vi "from string array.vi"(8 "error in (no error)":errorcluster, 9 "String Array":string[][](array[string]), 10 "version":string, 11 "module configuration in":refnum<class "Daqmx Module configuration.lvclass">) -> (0 "error out":errorcluster, 3 "module configuration out":refnum<class "Daqmx Module configuration.lvclass">)   [LabVIEW 2015, in "DAQmx Module Configuration.lvclass"]
uses:
  Daqmx Module configuration.lvclass
  Line.ctl
  <vilib>/NI/Tag Bus Module Framework/channel/TBM channel.lvclass
  Measurement Type.ctl
  Parameters.ctl
  <vilib>/NI/Tag Bus/tag/Data Type.ctl
  <vilib>/NI/Tag Bus Module Framework/channel/channel classification.ctl
  Daqmx Module configuration.lvclass/Daqmx Module configuration.ctl
  <vilib>/NI/Tag Bus/tag/tag descriptor.lvclass
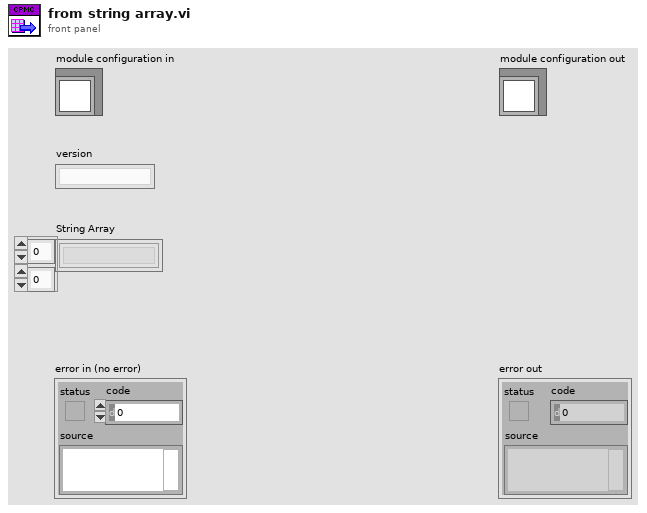
[diagram p1: front panel]
types:
  T1 = typedef "DAQmx Module Configuration.lvclass/Line.ctl" = cluster{"Channel Array":refnum<class "TBM channel.lvclass">[], "Physical Channel":string, "Measurement Type":T2, "Parameters":T3}
  T2 = typedef "DAQmx Module Configuration.lvclass/Measurement Type.ctl" = enum16{"Digital Input", "Digital Output", "Voltage Input", "Voltage Output", "Current Input", "Current Output", "RTD", "Thermocouple", "Strain", "PWM"}
  T3 = typedef "DAQmx Module Configuration.lvclass/Parameters.ctl" = cluster{"Digital Config":cluster{"Invert Lines?":bool}, "Voltage Config":cluster{"Maximum Value (V)":dbl, "Minimum Value (V)":dbl, "in terminal configuration (V)":i32, "out terminal configuration (V)":i32}, "Current Config":cluster{"Maximum Value (A)":dbl, "Minimum Value (A)":dbl, "shunt resistor location":i32, "input terminal configuration (C)":i32, "external shunt resistor value":dbl}, "RTD Config":cluster{"Maximum Value (°C)":dbl, "Minimum Value (°C)":dbl, "resistance configuration":i32, "r0":dbl, "current excitation value":dbl, "rtd type":i32, "current excitation source":i32}, "Thermocouple Config":cluster{"Minimum Value (C)":dbl, "Maximum Value (C)":dbl, "thermocouple type":i32, "cjc source":i32, "cjc value":dbl}, "Strain Config":cluster{"Maximum Value":dbl, "Minimum Value":dbl, "bridge information":cluster{"strain configuration":i32, "lead wire resistance":dbl, "initial bridge voltage":dbl, "voltage excitation source":i32, "voltage excitation value":dbl}, "strain gage information":cluster{"gage factor":dbl, "nominal gage resistance":dbl, "poisson ratio":dbl}}, "PWM Config":cluster{"Idle State":bool}}
  T4 = typedef "TBM channel.lvclass/channel classification.ctl" = enum16{"input data", "output data", "processing parameter", "processing result"}
  T5 = typedef "tag bus.lvlib/tag descriptor.lvclass/Data Type.ctl" = enum16{"Double", "Single", "I64", "I32", "I16", "I8", "U64", "U32", "U16", "U8", "Boolean", "String", "Array of Double", "Array of Single", "Array of I64", "Array of I32", "Array of I16", "Array of I8", "Array of U64", "Array of U32", "Array of U16", "Array of U8", "Array of Boolean", "Array of String"}
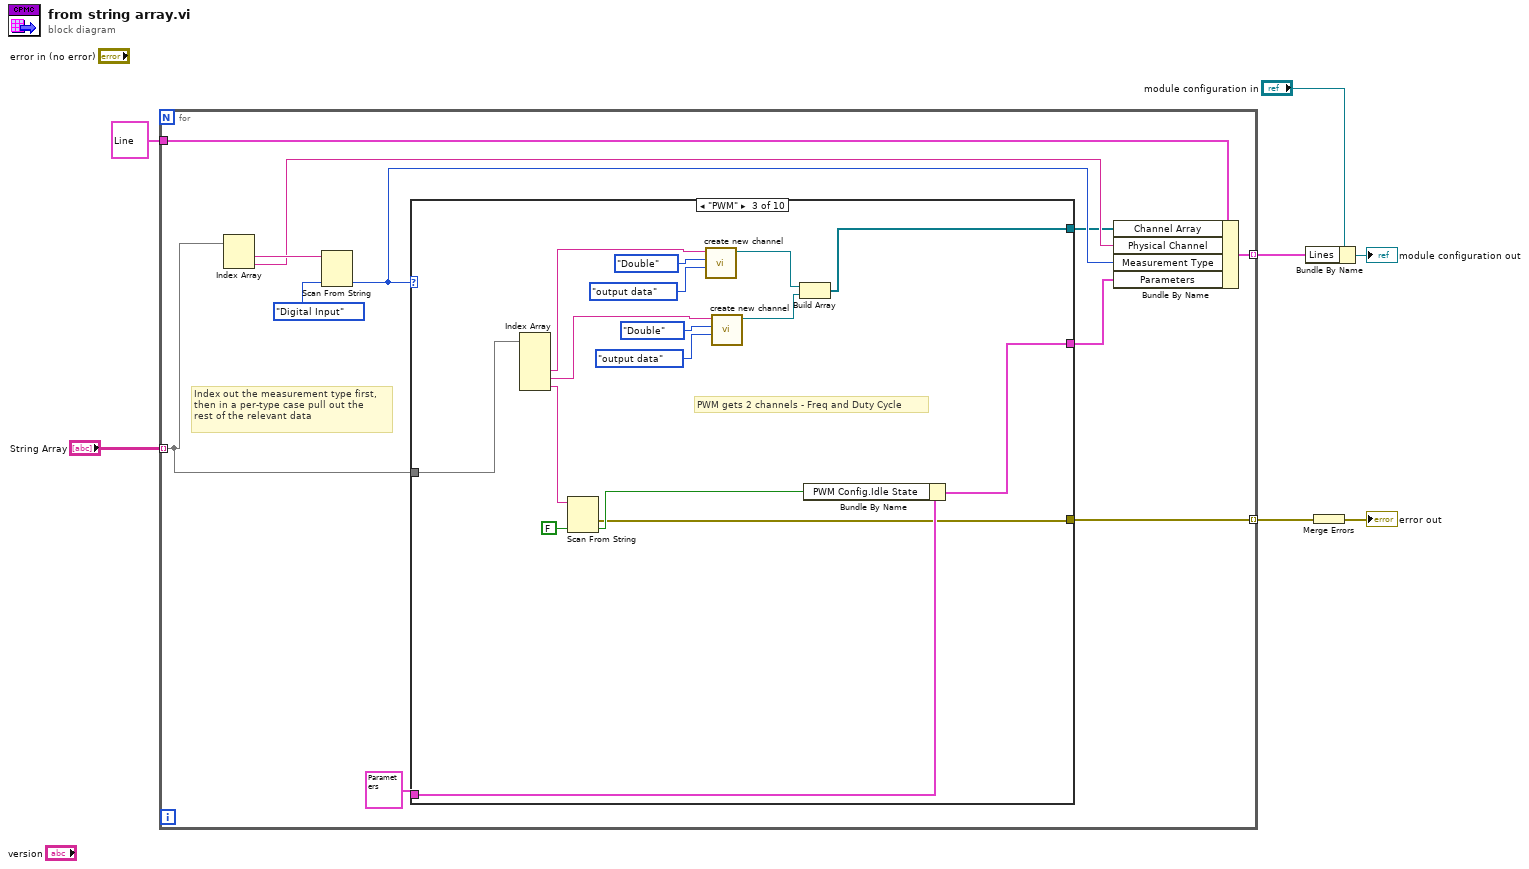
[diagram p0: block diagram]
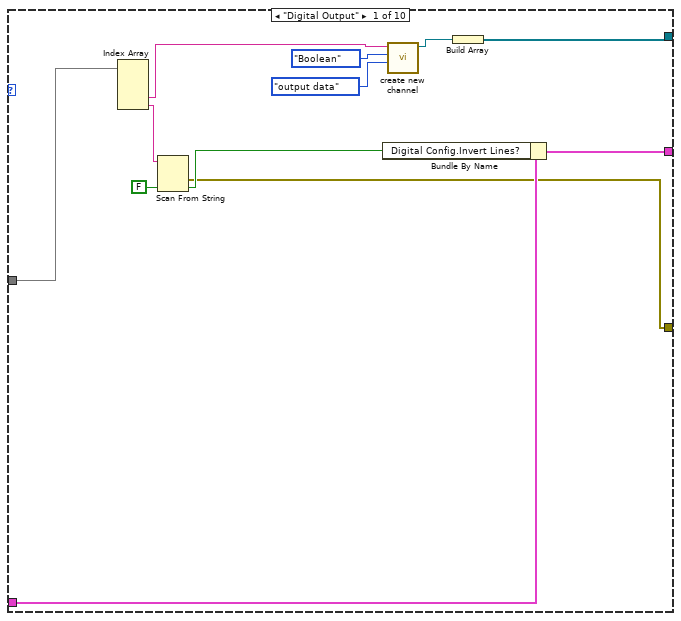
[diagram p2: hidden frame]
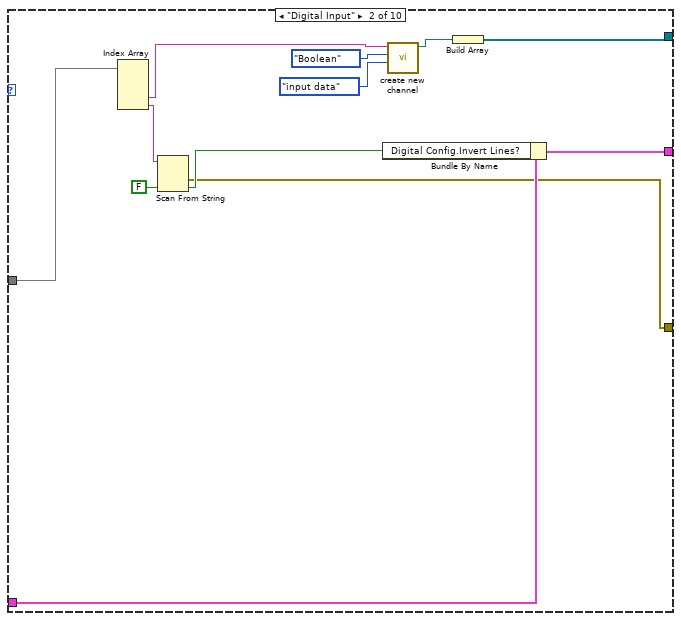
[diagram p3: hidden frame]
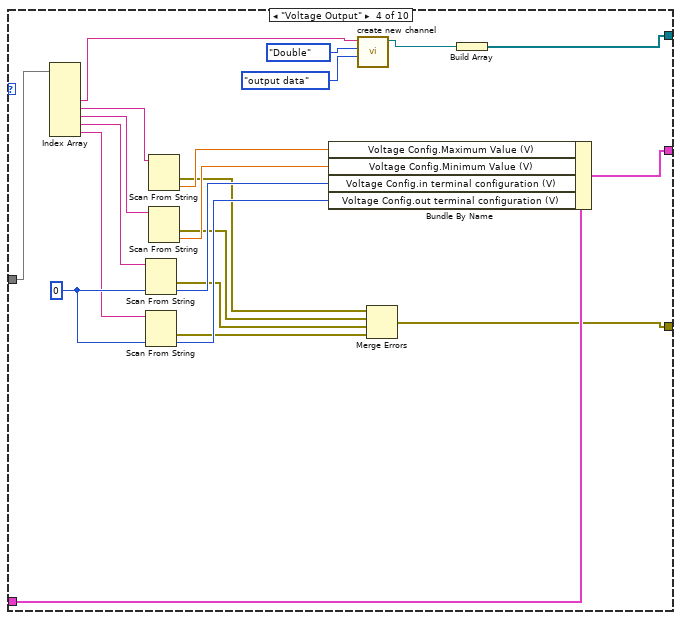
[diagram p4: hidden frame]
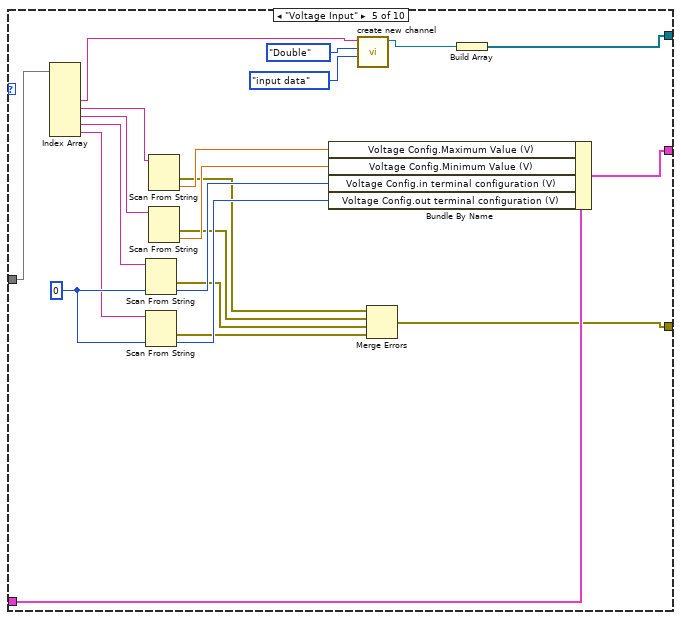
[diagram p5: hidden frame]
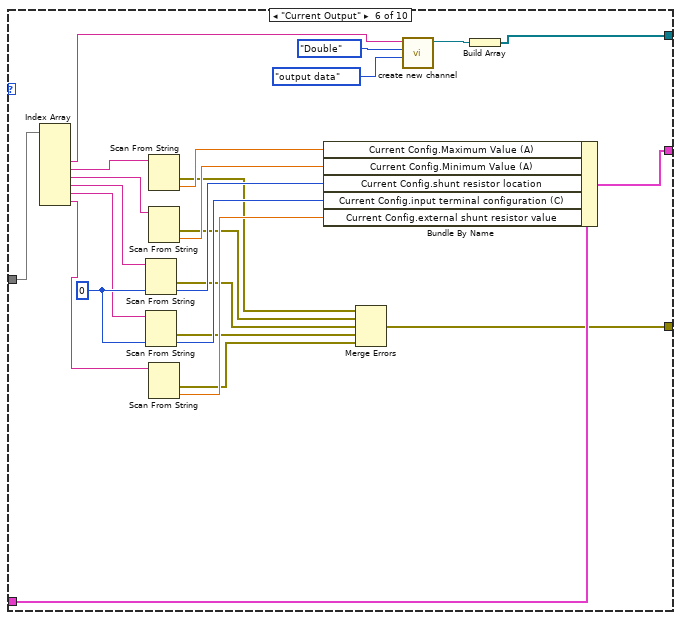
[diagram p6: hidden frame]
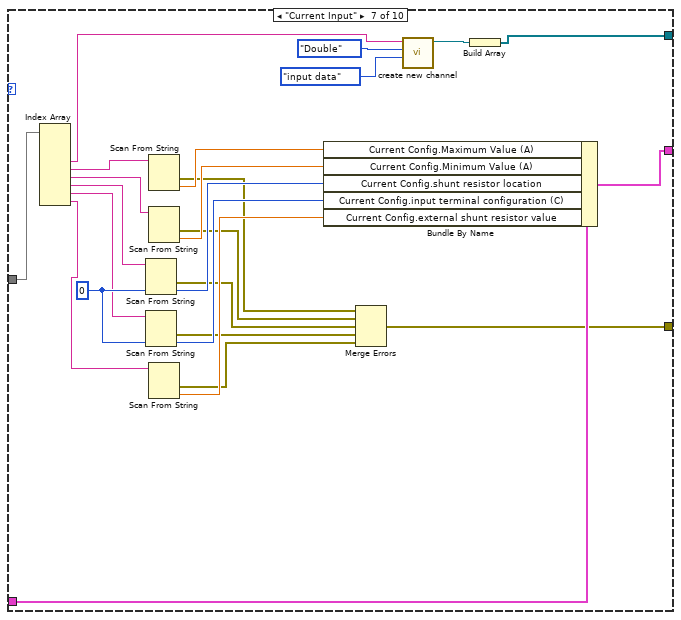
[diagram p7: hidden frame]
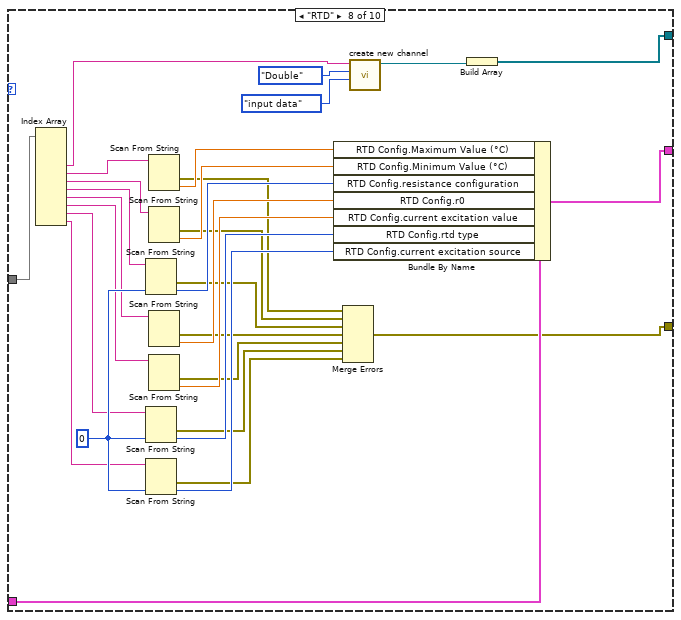
[diagram p8: hidden frame]
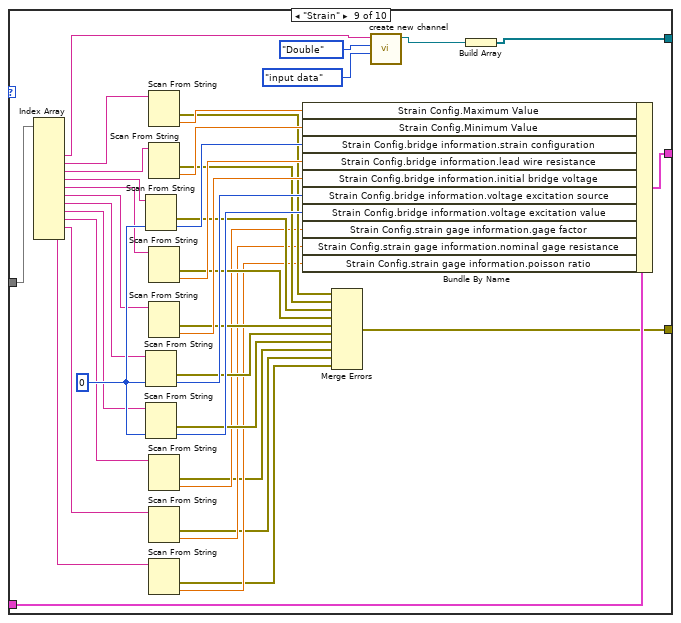
[diagram p9: hidden frame]
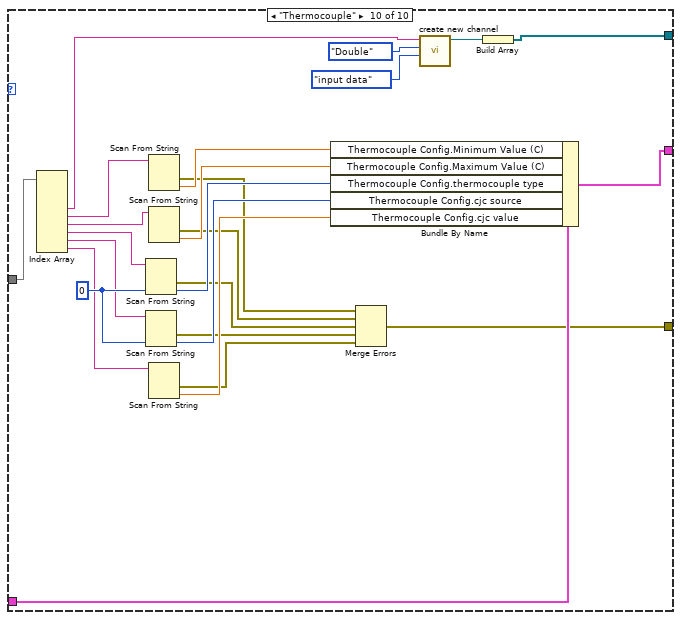
[diagram p10: hidden frame]
diagram:
  n1 = for {
    tunnel: "String Array" -> [w10] mode=indexing
    tunnel: T1 {"Channel Array"=[], "Physical Channel"="", "Measurement Type"=enum."Digital Input", "Parameters"={"Digital Config"={"Invert Lines?"=FALSE}, "Voltage Config"={"Maximum Value (V)"=5.0, "Minimum Value (V)"=-5.0, "in terminal configuration (V)"=-1, "out terminal configuration (V)"=-1}, "Current Config"={"Maximum Value (A)"=0.02, "Minimum Value (A)"=0.0, "shunt resistor location"=-1, "input terminal configuration (C)"=-1, "external shunt resistor value"=249.0}, "RTD Config"={"Maximum Value (°C)"=100.0, "Minimum Value (°C)"=0.0, "resistance configuration"=2, "r0"=100.0, "current excitation value"=0.0025, "rtd type"=10137, "current excitation source"=10167}, "Thermocouple Config"={"Minimum Value (C)"=0.0, "Maximum Value (C)"=100.0, "thermocouple type"=10072, "cjc source"=10116, "cjc value"=25.0}, "Strain Config"={"Maximum Value"=0.001, "Minimum Value"=-0.001, "bridge information"={"strain configuration"=10183, "lead wire resistance"=0.0, "initial bridge voltage"=0.0, "voltage excitation source"=10200, "voltage excitation value"=2.5}, "strain gage information"={"gage factor"=2.0, "nominal gage resistance"=350.0, "poisson ratio"=0.3}}, "PWM Config"={"Idle State"=FALSE}}} ("Line") -> [w18]
    tunnel: [w17] -> w4 mode=indexing
    tunnel: [w12] -> w2 mode=indexing
    # "Index out the measurement type first,\nthen in a per-type case pull out the\nrest of the relevant data"
    n2 = Index Array(array=w10) -> (element #1=w11:string, element #2=w9:string)  [unwired: 2 in]
    n3 = Scan From String(input string=w11, default 1=Measurement_Type."Digital Input" ("Measurement Type")) -> (output 1=w13:T2)  [unwired: 3 in, 3 out]
    n4 = case shown="\"PWM\"" w13 {
      tunnel: T3 {"Digital Config"={"Invert Lines?"=FALSE}, "Voltage Config"={"Maximum Value (V)"=5.0, "Minimum Value (V)"=-5.0, "in terminal configuration (V)"=-1, "out terminal configuration (V)"=-1}, "Current Config"={"Maximum Value (A)"=0.02, "Minimum Value (A)"=0.0, "shunt resistor location"=-1, "input terminal configuration (C)"=-1, "external shunt resistor value"=249.0}, "RTD Config"={"Maximum Value (°C)"=100.0, "Minimum Value (°C)"=0.0, "resistance configuration"=2, "r0"=100.0, "current excitation value"=0.0025, "rtd type"=10137, "current excitation source"=10167}, "Thermocouple Config"={"Minimum Value (C)"=0.0, "Maximum Value (C)"=100.0, "thermocouple type"=10072, "cjc source"=10116, "cjc value"=25.0}, "Strain Config"={"Maximum Value"=0.001, "Minimum Value"=-0.001, "bridge information"={"strain configuration"=10183, "lead wire resistance"=0.0, "initial bridge voltage"=0.0, "voltage excitation source"=10200, "voltage excitation value"=2.5}, "strain gage information"={"gage factor"=2.0, "nominal gage resistance"=350.0, "poisson ratio"=0.3}}, "PWM Config"={"Idle State"=FALSE}} ("Parameters") -> [w30 w42 w58 w80 w102 w127 w152 w183 w223 w248]
      tunnel: [w29 w41 w57 w79 w101 w126 w151 w182 w222 w247] -> w14
      tunnel: [w26 w38 w54 w69 w91 w114 w139 w166 w206 w236] -> w12
      tunnel: w10 -> [w23 w35 w51 w64 w86 w109 w134 w160 w195 w230]
      tunnel: [w20 w32 w46 w65 w87 w110 w135 w161 w196 w231] -> w8
      frame "Digital Output" {
        n5 = Index Array(array=w23) -> (element #3=w22:string, element #4=w19:string)  [unwired: 4 in, 2 out]
        n6 = Scan From String(input string=w19, default 1=FALSE ("Digital Config.Invert Lines?")) -> (error out=w26:errorcluster, output 1=w27:bool)  [unwired: 3 in, 2 out]
        n7 = Bundle By Name(cluster=w30, "Digital Config.Invert Lines?"=w27) -> (w29:T3)
        n8 = call <vilib>:"create new channel.vi"("channel classification"=channel_classification."output data", "data type"=Data_Type."Boolean", "channel name"=w22) -> ("channel"=w21:refnum<class "TBM channel.lvclass">)  [unwired: 8 in]
        n9 = Build Array(w21) -> (w20:refnum<class "TBM channel.lvclass">[])
      }
      frame "Digital Input" {
        n10 = Index Array(array=w35) -> (element #3=w34:string, element #4=w31:string)  [unwired: 4 in, 2 out]
        n11 = Scan From String(input string=w31, default 1=FALSE ("Digital Config.Invert Lines?")) -> (error out=w38:errorcluster, output 1=w39:bool)  [unwired: 3 in, 2 out]
        n12 = Bundle By Name(cluster=w42, "Digital Config.Invert Lines?"=w39) -> (w41:T3)
        n13 = call <vilib>:"create new channel.vi"("channel classification"=channel_classification."input data", "data type"=Data_Type."Boolean", "channel name"=w34) -> ("channel"=w33:refnum<class "TBM channel.lvclass">)  [unwired: 8 in]
        n14 = Build Array(w33) -> (w32:refnum<class "TBM channel.lvclass">[])
      }
      frame "PWM" {
        # "PWM gets 2 channels - Freq and Duty Cycle"
        n15 = Index Array(array=w51) -> (element #3=w45:string, element #4=w44:string, element #5=w43:string)  [unwired: 5 in, 2 out]
        n16 = Scan From String(input string=w43, default 1=FALSE ("Digital Config.Invert Lines?")) -> (error out=w54:errorcluster, output 1=w55:bool)  [unwired: 3 in, 2 out]
        n17 = call <vilib>:"create new channel.vi"("channel classification"=channel_classification."output data", "data type"=Data_Type."Double", "channel name"=w45) -> ("channel"=w48:refnum<class "TBM channel.lvclass">)  [unwired: 8 in]
        n18 = call <vilib>:"create new channel.vi"("channel classification"=channel_classification."output data", "data type"=Data_Type."Double", "channel name"=w44) -> ("channel"=w47:refnum<class "TBM channel.lvclass">)  [unwired: 8 in]
        n19 = Build Array(w48, w47) -> (w46:refnum<class "TBM channel.lvclass">[])
        n20 = Bundle By Name(cluster=w58, "PWM Config.Idle State"=w55) -> (w57:T3)
      }
      frame "Voltage Output" {
        w78 = 0 ("Voltage Config.out terminal configuration (V)")
        n21 = Index Array(array=w64) -> (element #3=w63:string, element #4=w62:string, element #5=w61:string, element #6=w60:string, element #7=w59:string)  [unwired: 7 in, 2 out]
        n22 = Scan From String(input string=w60, default 1=w78) -> (error out=w71:errorcluster, output 1=w76:i32)  [unwired: 3 in, 2 out]
        n23 = Scan From String(input string=w59, default 1=w78) -> (error out=w70:errorcluster, output 1=w77:i32)  [unwired: 3 in, 2 out]
        n24 = Scan From String(input string=w62) -> (error out=w73:errorcluster, output 1=w74:dbl)  [unwired: 4 in, 2 out]
        n25 = Scan From String(input string=w61) -> (error out=w72:errorcluster, output 1=w75:dbl)  [unwired: 4 in, 2 out]
        n26 = Bundle By Name(cluster=w80, "Voltage Config.Maximum Value (V)"=w74, "Voltage Config.Minimum Value (V)"=w75, "Voltage Config.in terminal configuration (V)"=w76, "Voltage Config.out terminal configuration (V)"=w77) -> (w79:T3)
        n27 = call <vilib>:"create new channel.vi"("channel classification"=channel_classification."output data", "data type"=Data_Type."Double", "channel name"=w63) -> ("channel"=w66:refnum<class "TBM channel.lvclass">)  [unwired: 8 in]
        n28 = Merge Errors(w73, w72, w71, w70) -> (w69:errorcluster)
        n29 = Build Array(w66) -> (w65:refnum<class "TBM channel.lvclass">[])
      }
      frame "Voltage Input" {
        w100 = 0 ("Voltage Config.out terminal configuration (V)")
        n30 = Index Array(array=w86) -> (element #3=w85:string, element #4=w84:string, element #5=w83:string, element #6=w82:string, element #7=w81:string)  [unwired: 7 in, 2 out]
        n31 = Scan From String(input string=w82, default 1=w100) -> (error out=w93:errorcluster, output 1=w98:i32)  [unwired: 3 in, 2 out]
        n32 = Scan From String(input string=w81, default 1=w100) -> (error out=w92:errorcluster, output 1=w99:i32)  [unwired: 3 in, 2 out]
        n33 = Scan From String(input string=w84) -> (error out=w95:errorcluster, output 1=w96:dbl)  [unwired: 4 in, 2 out]
        n34 = Scan From String(input string=w83) -> (error out=w94:errorcluster, output 1=w97:dbl)  [unwired: 4 in, 2 out]
        n35 = Bundle By Name(cluster=w102, "Voltage Config.Maximum Value (V)"=w96, "Voltage Config.Minimum Value (V)"=w97, "Voltage Config.in terminal configuration (V)"=w98, "Voltage Config.out terminal configuration (V)"=w99) -> (w101:T3)
        n36 = call <vilib>:"create new channel.vi"("channel classification"=channel_classification."input data", "data type"=Data_Type."Double", "channel name"=w85) -> ("channel"=w88:refnum<class "TBM channel.lvclass">)  [unwired: 8 in]
        n37 = Merge Errors(w95, w94, w93, w92) -> (w91:errorcluster)
        n38 = Build Array(w88) -> (w87:refnum<class "TBM channel.lvclass">[])
      }
      frame "Current Output" {
        w125 = 0 ("Voltage Config.out terminal configuration (V)")
        n39 = Index Array(array=w109) -> (element #3=w108:string, element #4=w107:string, element #5=w106:string, element #6=w105:string, element #7=w104:string, element #8=w103:string)  [unwired: 8 in, 2 out]
        n40 = Scan From String(input string=w105, default 1=w125) -> (error out=w117:errorcluster, output 1=w123:i32)  [unwired: 3 in, 2 out]
        n41 = Scan From String(input string=w104, default 1=w125) -> (error out=w116:errorcluster, output 1=w124:i32)  [unwired: 3 in, 2 out]
        n42 = Scan From String(input string=w107) -> (error out=w119:errorcluster, output 1=w121:dbl)  [unwired: 4 in, 2 out]
        n43 = Scan From String(input string=w106) -> (error out=w118:errorcluster, output 1=w122:dbl)  [unwired: 4 in, 2 out]
        n44 = Scan From String(input string=w103) -> (error out=w115:errorcluster, output 1=w120:dbl)  [unwired: 4 in, 2 out]
        n45 = Bundle By Name(cluster=w127, "Current Config.Maximum Value (A)"=w121, "Current Config.Minimum Value (A)"=w122, "Current Config.shunt resistor location"=w123, "Current Config.input terminal configuration (C)"=w124, "Current Config.external shunt resistor value"=w120) -> (w126:T3)
        n46 = Merge Errors(w119, w118, w117, w116, w115) -> (w114:errorcluster)
        n47 = call <vilib>:"create new channel.vi"("channel classification"=channel_classification."output data", "data type"=Data_Type."Double", "channel name"=w108) -> ("channel"=w111:refnum<class "TBM channel.lvclass">)  [unwired: 8 in]
        n48 = Build Array(w111) -> (w110:refnum<class "TBM channel.lvclass">[])
      }
      frame "Current Input" {
        w150 = 0 ("Voltage Config.out terminal configuration (V)")
        n49 = Index Array(array=w134) -> (element #3=w133:string, element #4=w132:string, element #5=w131:string, element #6=w130:string, element #7=w129:string, element #8=w128:string)  [unwired: 8 in, 2 out]
        n50 = Scan From String(input string=w130, default 1=w150) -> (error out=w142:errorcluster, output 1=w148:i32)  [unwired: 3 in, 2 out]
        n51 = Scan From String(input string=w129, default 1=w150) -> (error out=w141:errorcluster, output 1=w149:i32)  [unwired: 3 in, 2 out]
        n52 = Scan From String(input string=w132) -> (error out=w144:errorcluster, output 1=w146:dbl)  [unwired: 4 in, 2 out]
        n53 = Scan From String(input string=w131) -> (error out=w143:errorcluster, output 1=w147:dbl)  [unwired: 4 in, 2 out]
        n54 = Scan From String(input string=w128) -> (error out=w140:errorcluster, output 1=w145:dbl)  [unwired: 4 in, 2 out]
        n55 = Bundle By Name(cluster=w152, "Current Config.Maximum Value (A)"=w146, "Current Config.Minimum Value (A)"=w147, "Current Config.shunt resistor location"=w148, "Current Config.input terminal configuration (C)"=w149, "Current Config.external shunt resistor value"=w145) -> (w151:T3)
        n56 = Merge Errors(w144, w143, w142, w141, w140) -> (w139:errorcluster)
        n57 = call <vilib>:"create new channel.vi"("channel classification"=channel_classification."input data", "data type"=Data_Type."Double", "channel name"=w133) -> ("channel"=w136:refnum<class "TBM channel.lvclass">)  [unwired: 8 in]
        n58 = Build Array(w136) -> (w135:refnum<class "TBM channel.lvclass">[])
      }
      frame "RTD" {
        w174 = 0 ("Voltage Config.out terminal configuration (V)")
        n59 = Index Array(array=w160) -> (element #3=w163:string, element #4=w159:string, element #5=w158:string, element #6=w157:string, element #7=w156:string, element #8=w155:string, element #9=w154:string, element #10=w153:string)  [unwired: 10 in, 2 out]
        n60 = Scan From String(input string=w157, default 1=w174) -> (error out=w171:errorcluster, output 1=w180:i32)  [unwired: 3 in, 2 out]
        n61 = Scan From String(input string=w154, default 1=w174) -> (error out=w168:errorcluster, output 1=w176:i32)  [unwired: 3 in, 2 out]
        n62 = Scan From String(input string=w153, default 1=w174) -> (error out=w167:errorcluster, output 1=w175:i32)  [unwired: 3 in, 2 out]
        n63 = Scan From String(input string=w159) -> (error out=w173:errorcluster, output 1=w178:dbl)  [unwired: 4 in, 2 out]
        n64 = Scan From String(input string=w158) -> (error out=w172:errorcluster, output 1=w179:dbl)  [unwired: 4 in, 2 out]
        n65 = Scan From String(input string=w156) -> (error out=w170:errorcluster, output 1=w181:dbl)  [unwired: 4 in, 2 out]
        n66 = Scan From String(input string=w155) -> (error out=w169:errorcluster, output 1=w177:dbl)  [unwired: 4 in, 2 out]
        n67 = Bundle By Name(cluster=w183, "RTD Config.Maximum Value (°C)"=w178, "RTD Config.Minimum Value (°C)"=w179, "RTD Config.resistance configuration"=w180, "RTD Config.r0"=w181, "RTD Config.current excitation value"=w177, "RTD Config.rtd type"=w176, "RTD Config.current excitation source"=w175) -> (w182:T3)
        n68 = Merge Errors(w173, w172, w171, w170, w169, w168, w167) -> (w166:errorcluster)
        n69 = call <vilib>:"create new channel.vi"("channel classification"=channel_classification."input data", "data type"=Data_Type."Double", "channel name"=w163) -> ("channel"=w162:refnum<class "TBM channel.lvclass">)  [unwired: 8 in]
        n70 = Build Array(w162) -> (w161:refnum<class "TBM channel.lvclass">[])
      }
      frame "Strain" {
        w214 = 0 ("Voltage Config.out terminal configuration (V)")
        n71 = Index Array(array=w195) -> (element #3=w194:string, element #4=w193:string, element #5=w192:string, element #6=w191:string, element #7=w190:string, element #8=w189:string, element #9=w188:string, element #10=w187:string, element #11=w186:string, element #12=w185:string, element #13=w184:string)  [unwired: 13 in, 2 out]
        n72 = Scan From String(input string=w191, default 1=w214) -> (error out=w211:errorcluster, output 1=w220:i32)  [unwired: 3 in, 2 out]
        n73 = Scan From String(input string=w188, default 1=w214) -> (error out=w208:errorcluster, output 1=w216:i32)  [unwired: 3 in, 2 out]
        n74 = Scan From String(input string=w187, default 1=w214) -> (error out=w207:errorcluster, output 1=w215:i32)  [unwired: 3 in, 2 out]
        n75 = Scan From String(input string=w193) -> (error out=w213:errorcluster, output 1=w218:dbl)  [unwired: 4 in, 2 out]
        n76 = Scan From String(input string=w192) -> (error out=w212:errorcluster, output 1=w219:dbl)  [unwired: 4 in, 2 out]
        n77 = Scan From String(input string=w190) -> (error out=w210:errorcluster, output 1=w221:dbl)  [unwired: 4 in, 2 out]
        n78 = Scan From String(input string=w189) -> (error out=w209:errorcluster, output 1=w217:dbl)  [unwired: 4 in, 2 out]
        n79 = Scan From String(input string=w186) -> (error out=w202:errorcluster, output 1=w205:dbl)  [unwired: 4 in, 2 out]
        n80 = Scan From String(input string=w185) -> (error out=w201:errorcluster, output 1=w204:dbl)  [unwired: 4 in, 2 out]
        n81 = Scan From String(input string=w184) -> (error out=w200:errorcluster, output 1=w203:dbl)  [unwired: 4 in, 2 out]
        n82 = Bundle By Name(cluster=w223, "Strain Config.Maximum Value"=w218, "Strain Config.Minimum Value"=w219, "Strain Config.bridge information.strain configuration"=w220, "Strain Config.bridge information.lead wire resistance"=w221, "Strain Config.bridge information.initial bridge voltage"=w217, "Strain Config.bridge information.voltage excitation source"=w216, "Strain Config.bridge information.voltage excitation value"=w215, "Strain Config.strain gage information.gage factor"=w205, "Strain Config.strain gage information.nominal gage resistance"=w204, "Strain Config.strain gage information.poisson ratio"=w203) -> (w222:T3)
        n83 = Merge Errors(w213, w212, w211, w210, w209, w208, w207, w202, w201, w200) -> (w206:errorcluster)
        n84 = call <vilib>:"create new channel.vi"("channel classification"=channel_classification."input data", "data type"=Data_Type."Double", "channel name"=w194) -> ("channel"=w197:refnum<class "TBM channel.lvclass">)  [unwired: 8 in]
        n85 = Build Array(w197) -> (w196:refnum<class "TBM channel.lvclass">[])
      }
      frame "Thermocouple" {
        w235 = 0 ("Voltage Config.out terminal configuration (V)")
        n86 = Index Array(array=w230) -> (element #3=w229:string, element #4=w228:string, element #5=w227:string, element #6=w226:string, element #7=w225:string, element #8=w224:string)  [unwired: 8 in, 2 out]
        n87 = Scan From String(input string=w226, default 1=w235) -> (error out=w239:errorcluster, output 1=w245:i32)  [unwired: 3 in, 2 out]
        n88 = Scan From String(input string=w225, default 1=w235) -> (error out=w238:errorcluster, output 1=w246:i32)  [unwired: 3 in, 2 out]
        n89 = Scan From String(input string=w228) -> (error out=w241:errorcluster, output 1=w243:dbl)  [unwired: 4 in, 2 out]
        n90 = Scan From String(input string=w227) -> (error out=w240:errorcluster, output 1=w244:dbl)  [unwired: 4 in, 2 out]
        n91 = Scan From String(input string=w224) -> (error out=w237:errorcluster, output 1=w242:dbl)  [unwired: 4 in, 2 out]
        n92 = Bundle By Name(cluster=w248, "Thermocouple Config.Minimum Value (C)"=w243, "Thermocouple Config.Maximum Value (C)"=w244, "Thermocouple Config.thermocouple type"=w245, "Thermocouple Config.cjc source"=w246, "Thermocouple Config.cjc value"=w242) -> (w247:T3)
        n93 = Merge Errors(w241, w240, w239, w238, w237) -> (w236:errorcluster)
        n94 = call <vilib>:"create new channel.vi"("channel classification"=channel_classification."input data", "data type"=Data_Type."Double", "channel name"=w229) -> ("channel"=w232:refnum<class "TBM channel.lvclass">)  [unwired: 8 in]
        n95 = Build Array(w232) -> (w231:refnum<class "TBM channel.lvclass">[])
      }
    }
    n96 = Bundle By Name(cluster=w18, "Channel Array"=w8, "Physical Channel"=w9, "Measurement Type"=w13, "Parameters"=w14) -> (w17:T1)
  }
  n97 = Bundle By Name(cluster="module configuration in", "Lines"=w4) -> (→"module configuration out":refnum<class "Daqmx Module configuration.lvclass">)
  n98 = Merge Errors(w2) -> (→"error out":errorcluster)
